vi "VIH HelpGen - Write HTML File - VI - Control Descriptions.vi"(4 "InstanceRef":string, 6 "Ctrl Dscr Params":T6, 7 "Save params":T1, 8 "error in":errorcluster, 9 "Table Templates":T7, 10 "HTML in":string, 11 "VI Reference":refnum<vi>) -> (0 "error out":errorcluster, 2 "HTML out":string, 3 "dup VI Reference":refnum<vi>)   [LabVIEW 2014]
doc: "::: VI Helpeks :::\nCopyright (c) 2000-2026 Konstantin Shifershteyn. All rights reserved."
uses:
  VIH HelpGen Typedef - Table Templates Cluster - VI Help.ctl
  VIH HelpGen Typedef - Cluster - Control Rule.ctl
  VIH HelpGen Typedef - Enum - Description Mode.ctl
  VIH HelpGen Typedef - Enum - Default,Enable,Disable.ctl
  VIH HelpGen Typedef - Cluster - Enum Value Info.ctl
panel:
  # "VI Helpeks\nCopyright (c) 2012-2026 Konstantin Shifershteyn"
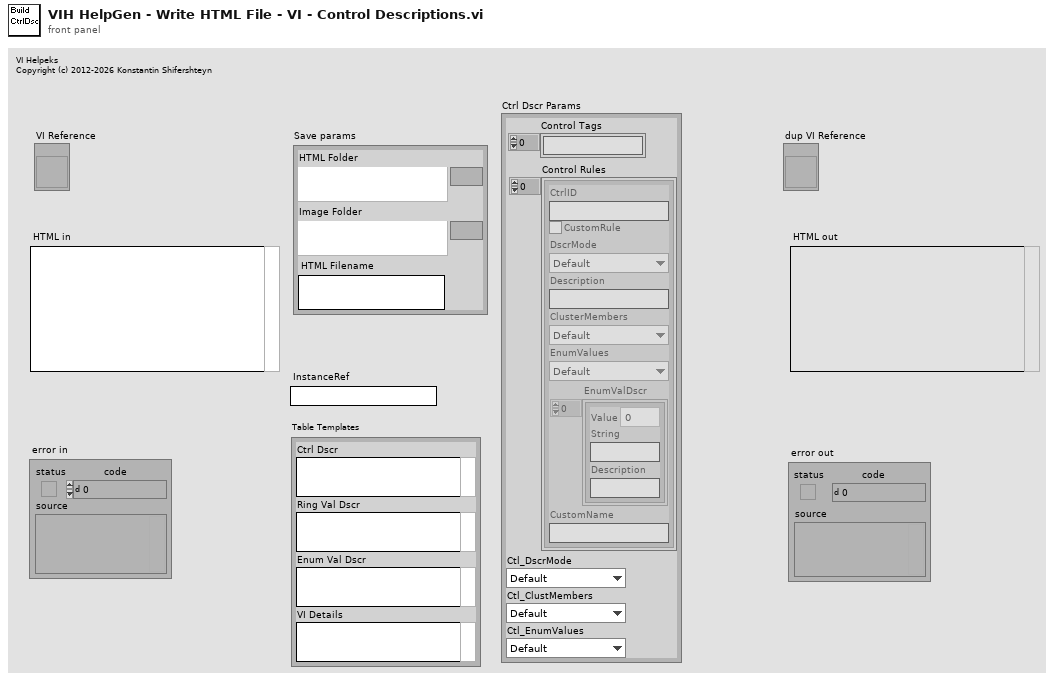
[diagram p1: front panel]
types:
  T1 = cluster{"HTML Folder":path, "Image Folder":path, "HTML Filename":string}
  T2 = typedef "VIH HelpGen Typedef - Cluster - Control Rule.ctl" = cluster{"CtrlID":string, "CustomRule":bool, "DscrMode":T3, "Description":string, "ClusterMembers":T4, "EnumValues":T4, "EnumValDscr":T5[], "CustomName":string}
  T3 = typedef "VIH HelpGen Typedef - Enum - Description Mode.ctl" = enum16{"Default", "Description", "Description1", "Description2", "Custom", "None"}
  T4 = typedef "VIH HelpGen Typedef - Enum - Default,Enable,Disable.ctl" = enum16{"Default", "Enable", "Disable"}
  T5 = typedef "VIH HelpGen Typedef - Cluster - Enum Value Info.ctl" = cluster{"Value":ext, "String":string, "Description":string}
  T6 = cluster{"Control Tags":string[], "Control Rules":T2[], "Ctl_DscrMode":T3, "Ctl_ClustMembers":T4, "Ctl_EnumValues":T4}
  T7 = typedef "VIH HelpGen Typedef - Table Templates Cluster - VI Help.ctl" = cluster{"Ctrl Dscr":string, "Ring Val Dscr":string, "Enum Val Dscr":string, "VI Details":string}
  T8 = typedef "VIH HelpGen Typedef - Control Terminal Attributes Cluster.ctl" = cluster{"Conpane Idx":i32, "Control":bool, "Wire Rule":enum16{"Invalid Wire Rule", "Required", "Recommended", "Optional", "Dynamic Dispatch"}}
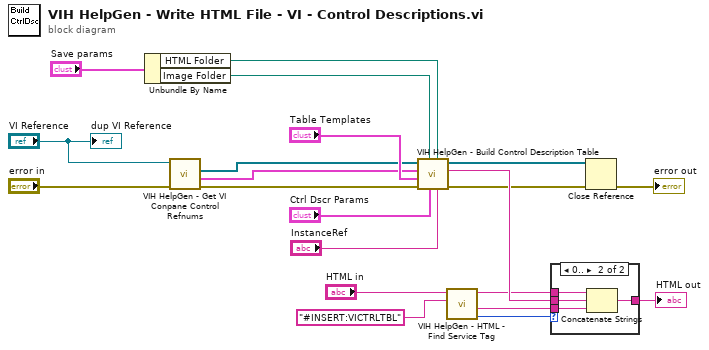
[diagram p0: block diagram]
diagram:
  n1 = Unbundle By Name("Save params") -> ("HTML Folder"=w2:path, "Image Folder"=w1:path)
  n2 = call "VIH HelpGen - Get VI Conpane Control Refnums.vi"("error in"="error in", "VI Reference"="VI Reference") -> ("error out"=w20:errorcluster, "Ctrl Attributes"=w7:T8[], "Conpane Ctrl Refnums"=w11:refnum<vi>[])  [unwired: 6 in, 1 out]
  n3 = call "VIH HelpGen - Build Control Description Table.vi"("InstanceRef"="InstanceRef", "HTML Folder"=w2, "Ctrl Dscr Params"="Ctrl Dscr Params", "Image Folder"=w1, "error in"=w20, "Table Templates"="Table Templates", "Ctrl Attributes"=w7, "Ctrl refnums"=w11) -> ("error out"=w9:errorcluster, "HTML out"=w19:string, "dup Ctrl refnums"=w10:refnum<vi>[])  [unwired: 1 in]
  n4 = call "VIH HelpGen - HTML - Find Service Tag.vi"("Tag name"="#INSERT:VICTRLTBL", "HTML in"="HTML in") -> ("Offset out"=w6:i32, "After"=w15:string, "Before"=w16:string)  [unwired: 6 in, 1 out]
  n5 = case shown="0.." w6 {
    tunnel: w19 -> [_ w26]
    tunnel: [w22 w25] -> w18
    tunnel: w16 -> [w22 w24]
    tunnel: w15 -> [_ w23]
    frame ..-1 {
    }
    frame 0.. {
      n6 = Concatenate Strings(w24, w26, w23) -> (w25:string)
    }
  }
  "HTML out" <- w18
  n7 = Close Reference(reference=w10, error in (no error)=w9) -> (error out=→"error out":errorcluster)
  "dup VI Reference" <- "VI Reference"
